vi "SC Fill Version List.vi"(4 "error in (no error)":errorcluster, 8 "others discarded?":bool=TRUE, 9 "others":string[](array[string]), 10 "keeps":string[](array[string]), 11 "list":refnum<vi>) -> (0 "error out":errorcluster)   [LabVIEW 2023]
doc: "Fills a one-column multicolumn listbox of SC Choose Version with commits: keeps (a check) first, then others in grey; when others discarded? is set they're the commits that choice discards, crossed out and struck through. Sizes the column to the list."
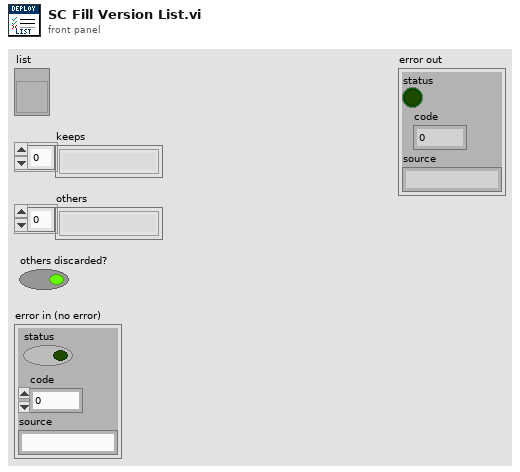
[diagram p1: front panel]
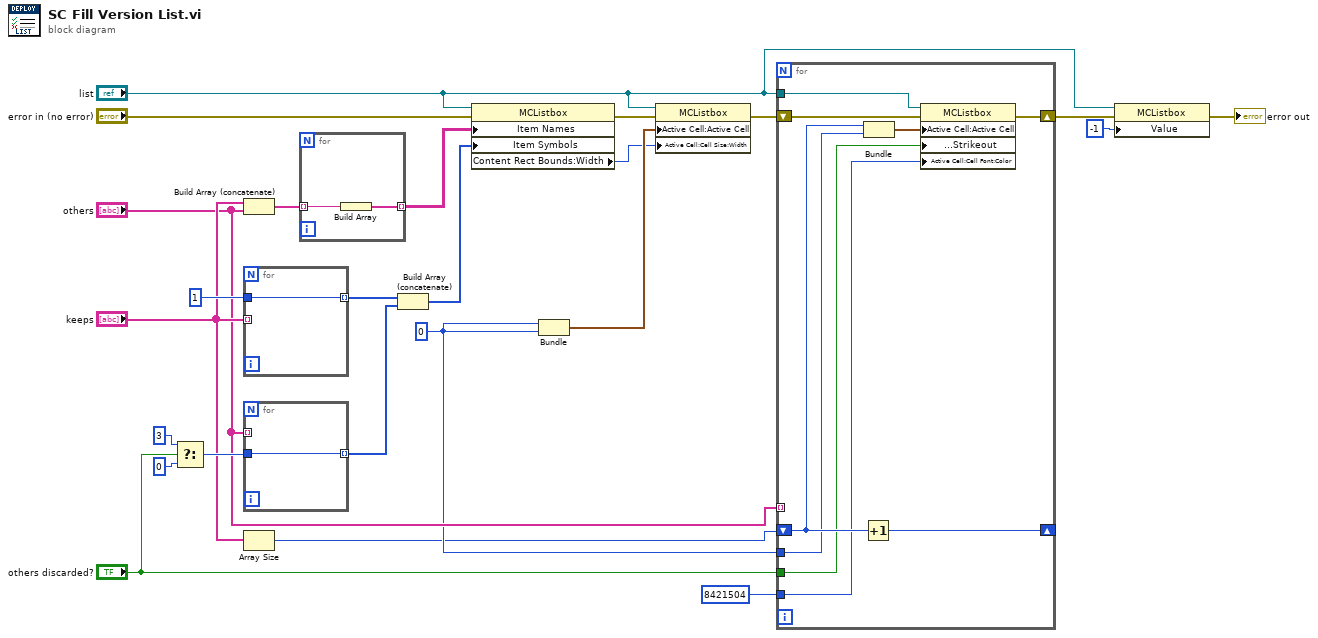
[diagram p0: block diagram]
diagram:
  w7 = 0
  n1 = Select(t=3, s="others discarded?", f=0) -> (s? t:f=w20:i32)
  n2 = Build Array (concatenate)("keeps", "others") -> (w24:string[])
  n3 = for {
    tunnel: "keeps" -> [_] mode=indexing
    tunnel: 1 -> [w25]
    tunnel: [w25] -> w19 mode=indexing
  }
  n4 = for {
    tunnel: "others" -> [_] mode=indexing
    tunnel: w20 -> [w26]
    tunnel: [w26] -> w18 mode=indexing
  }
  n5 = Array Size(array="keeps") -> (size(s)=w6:i32)
  n6 = for {
    tunnel: w24 -> [w28] mode=indexing
    tunnel: [w27] -> w16 mode=indexing
    n7 = Build Array(w28) -> (w27:string[])
  }
  n8 = Build Array (concatenate)(w19, w18) -> (w15:i32[])
  n9 = property class="MCListbox"(reference="list", error in="error in (no error)", "Item Names"=w16, "Item Symbols"=w15) -> (error out=w14:errorcluster, "Content Rect Bounds:Width"=w12:i32)  [unwired: 1 out]
  n10 = Bundle(w7, w7) -> (w13:cluster{i32, i32})  [unwired: 1 in]
  n11 = property class="MCListbox"(reference="list", error in=w14, "Active Cell:Active Cell"=w13, "Active Cell:Cell Size:Width"=w12) -> (error out=w5:errorcluster)  [unwired: 1 out]
  n12 = for {
    tunnel: "others" -> [_] mode=indexing
    tunnel: "list" -> [w34]
    tunnel: "others discarded?" -> [w31]
    tunnel: u32 8421504 -> [w30]
    tunnel: w7 -> [w35]
    shift-right: [w37] -> _
    shift-left: w6 -> [w36]
    shift-right: [w29] -> w3
    shift-left: w5 -> [w33]
    n13 = Increment(x=w36) -> (x+1=w37:i32)
    n14 = Bundle(w36, w35) -> (w32:cluster{i32, i32})  [unwired: 1 in]
    n15 = property class="MCListbox"(reference=w34, error in=w33, "Active Cell:Active Cell"=w32, "Active Cell:Cell Font:Strikeout"=w31, "Active Cell:Cell Font:Color"=w30) -> (error out=w29:errorcluster)  [unwired: 1 out]
  }
  n16 = property class="MCListbox"(reference="list", error in=w3, "Value"=-1) -> (error out=→"error out":errorcluster)  [unwired: 1 out]
